vi "support.read_and_free_string_at_address.vi"(6 "string_length":u64, 8 "error in (no error)":errorcluster, 11 "string_ptr":u64) -> (0 "error out":errorcluster, 3 "string":string)   [LabVIEW 2020, in "toml_edit.lvlib"]
uses:
  toml_edit.lvlib
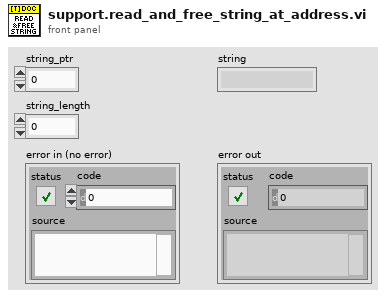
[diagram p1: front panel]
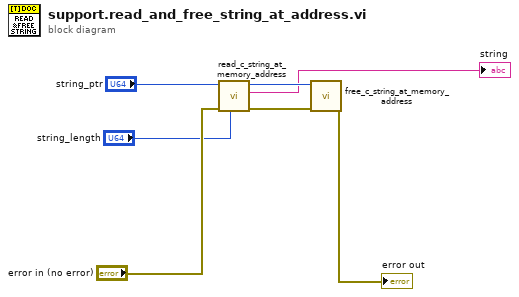
[diagram p0: block diagram]
diagram:
  n1 = call "read_c_string_at_memory_address.vi"("estimated bytes"="string_length", "error in (no error)"="error in (no error)", "memory_address"="string_ptr") -> ("error out"=w6:errorcluster, "string"=→"string":string, "memory_address out"=w5:u64)  [unwired: 6 in]
  n2 = call "free_c_string_at_memory_address.vi"("error in (no error)"=w6, "memory_address"=w5) -> ("error out"=→"error out":errorcluster)  [unwired: 9 in]
